vi "Register Job Event.vi"(11 "Job in":refnum<class "Job.lvclass">) -> (2 "Job Event Registration":refnum<event-registration>, 3 "Job out":refnum<class "Job.lvclass">)   [LabVIEW 2013, in "openCronJob.lvlib" / "Job.lvclass"]
uses:
  Job.lvclass
  JobReport/JobReport.lvclass
  Job Started -- cluster.ctl
  Job Update -- cluster.ctl
  Job.lvclass/Job.ctl
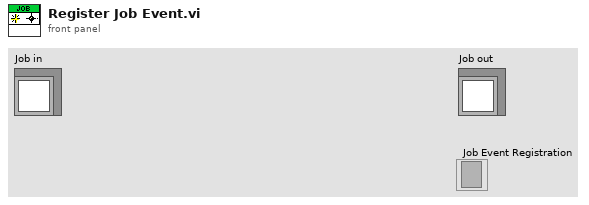
[diagram p1: front panel]
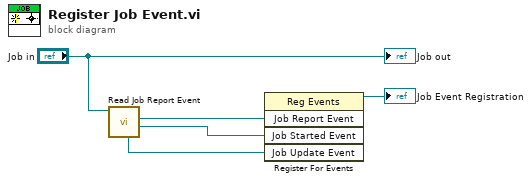
[diagram p0: block diagram]
diagram:
  n1 = call "Read Job Report Event.vi"("Job in"="Job in") -> ("Job Started Event"=w3:refnum<user-event>, "Job Report Event"=w4:refnum<user-event>, "Job Update Event"=w2:refnum<user-event>)  [unwired: 6 in, 2 out]
  n2 = register-events(w4, w3, w2) -> (reference out=→"Job Event Registration":refnum<event-registration>)  [unwired: 2 in, 1 out]
  "Job out" <- "Job in"
